vi "Round To Cents.vi"(11 "amount":dbl) -> (3 "rounded":dbl)   [LabVIEW 2020, in "Full Featured MCP Server.lvlib"]
doc: "Rounds an amount of money to two decimals."
uses:
  Full Featured MCP Server.lvlib
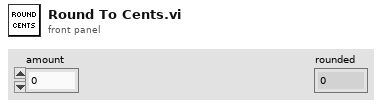
[diagram p1: front panel]
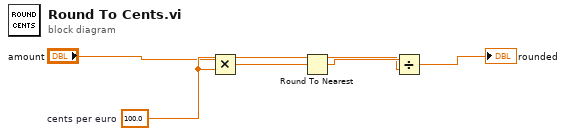
[diagram p0: block diagram]
diagram:
  w2 = 100.0  # cents per euro
  n1 = Multiply(x="amount", y=w2) -> (x*y=w3:dbl)
  n2 = Round To Nearest(number=w3) -> (nearest integer value=w4:dbl)
  n3 = Divide(x=w4, y=w2) -> (x/y=→"rounded":dbl)
